vi "RDV-addDataToMap2.vi"(7 "Add mod":string, 8 "error in (no error)":errorcluster, 9 "Data":T1[](array[typedef]), 10 "Names":string[](array[string]), 11 "RDV-Reflection_Data_viewer in":refnum<class "RDV-Reflection_Data_viewer.lvclass">) -> (0 "error out":errorcluster, 1 "Keys":string[](array[string]), 3 "RDV-Reflection_Data_viewer out":refnum<class "RDV-Reflection_Data_viewer.lvclass">)   [LabVIEW 2020, in "RDV-Reflection_Data_viewer.lvclass"]
doc: "Adds data clusters to the viewer's data map, with keys built from the file names and Add mod. Returns the keys."
uses:
  RDV-Reflection_Data_viewer.lvclass
  Reflector/RFH-common_data_format.ctl
  RDV-DATA_MAP_CLUST.ctl
  RDV-Reflection_Data_viewer.lvclass/RDV-Reflection_Data_viewer.ctl
  Reflector/RFH-Reflection_File_Handler.lvlib
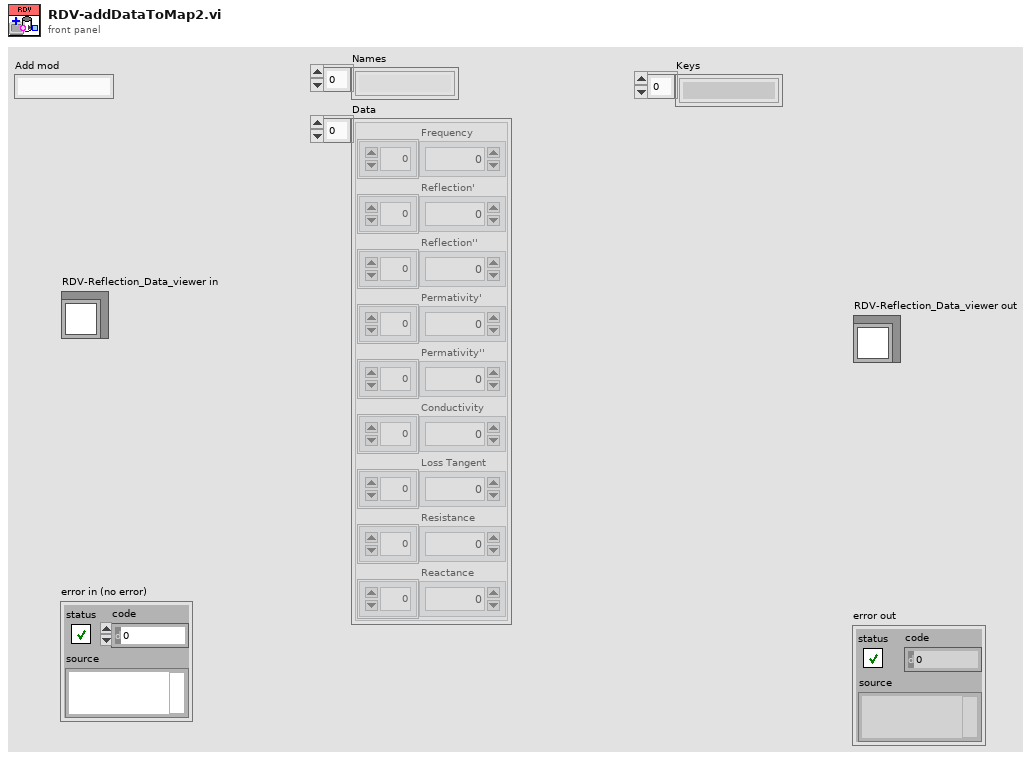
[diagram p1: front panel]
types:
  T1 = typedef "RFH-Reflection_File_Handler.lvlib/RFH-common_data_format.ctl" = cluster{"Frequency":dbl[], "Reflection'":dbl[], "Reflection''":dbl[], "Permativity'":dbl[], "Permativity''":dbl[], "Conductivity":dbl[], "Loss Tangent":dbl[], "Resistance":dbl[], "Reactance":dbl[]}
  T2 = typedef "RDV-Reflection_Data_viewer.lvclass/RDV-DATA_MAP_CLUST.ctl" = cluster{"filename w/ ext":string, "Common Format":T1}
  T3 = typedef "RDV-Reflection_Data_viewer.lvclass/RDV-DATA_MAP.ctl" = map{string, T2}
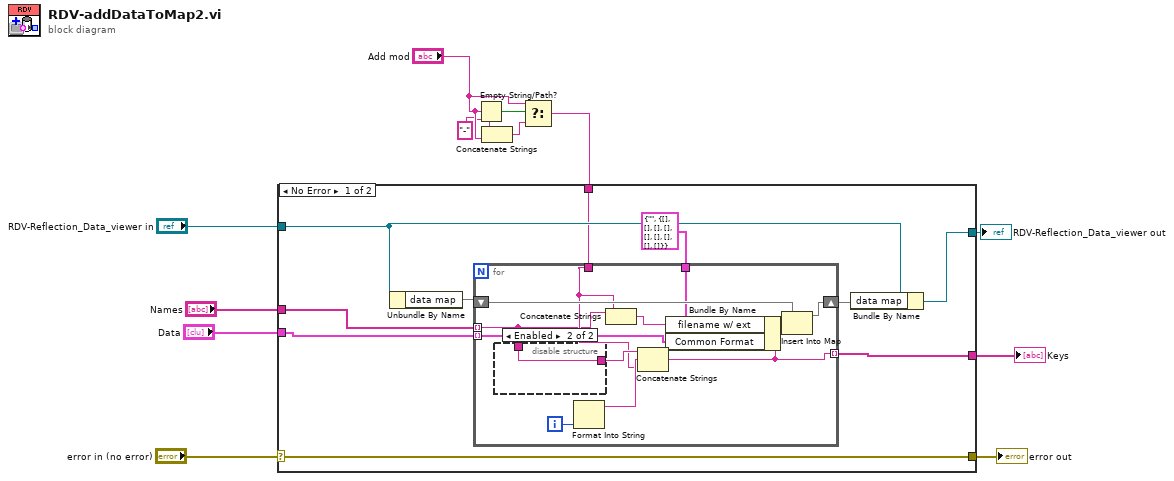
[diagram p0: block diagram]
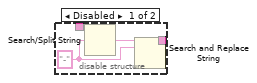
[diagram p2: hidden frame]
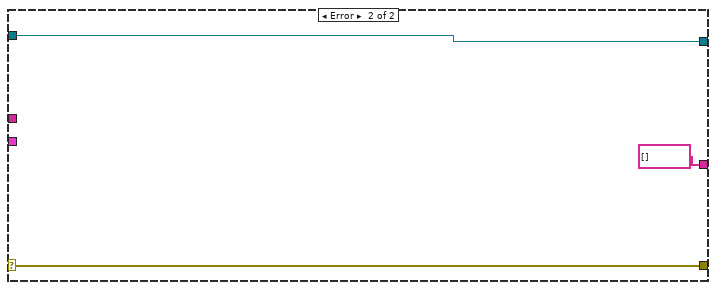
[diagram p3: hidden frame]
diagram:
  n1 = Empty String/Path?(string/path="Add mod") -> (empty?=w6:bool)
  n2 = Concatenate Strings("-" ("string"), "Add mod") -> (w8:string)
  n3 = Select(t="Add mod", s=w6, f=w8) -> (s? t:f=w2:string)
  n4 = case shown="No Error" "error in (no error)" {
    selector: "error in (no error)" -> [w22 w42]
    tunnel: [w22 w42] -> w11
    tunnel: [w16 w41] -> w9
    tunnel: "RDV-Reflection_Data_viewer in" -> [w15 w41]
    tunnel: "Data" -> [w17 _]
    tunnel: "Names" -> [w18 _]
    tunnel: w2 -> [w14 _]
    tunnel: [w13 string[] []] -> w1
    frame No Error {
      n5 = Unbundle By Name(w15) -> ("data map"=w21:T3)
      n6 = for {
        tunnel: w18 -> [w27] mode=indexing
        tunnel: w17 -> [w23] mode=indexing
        shift-right: [w33] -> w20
        shift-left: w21 -> [w34]
        tunnel: [w29] -> w13 mode=indexing
        tunnel: w14 -> [w28]
        tunnel: T2 {"filename w/ ext"="", "Common Format"={"Frequency"=[], "Reflection'"=[], "Reflection''"=[], "Permativity'"=[], "Permativity''"=[], "Conductivity"=[], "Loss Tangent"=[], "Resistance"=[], "Reactance"=[]}} ("map  data") -> [w26]
        i -> [w32]
        n7 = disable-structure shown="Enabled" {
          disable-tunnel: [w36 w39] -> w31
          disable-tunnel: w27 -> [w35 w39]
          frame Disabled {
            w37 = "-" ("search string/char (-)")
            n8 = Search/Split String(string=w35, search string/char (-)=w37) -> (match + rest of string=w38:string)  [unwired: 1 in, 2 out]
            n9 = Search and Replace String(input string=w38, search string=w37) -> (result string=w36:string)  [unwired: 6 in, 3 out]
          }
          frame Enabled {
          }
        }
        n10 = Format Into String(w32) -> (resulting string=w30:string)  [unwired: 3 in, 1 out]
        n11 = Concatenate Strings(w27, w28) -> (w24:string)
        n12 = Concatenate Strings(w31, w30, w28) -> (w29:string)
        n13 = Bundle By Name(cluster=w26, "filename w/ ext"=w24, "Common Format"=w23) -> (w25:T2)
        n14 = Insert Into Map(map in=w34, key=w29, value=w25) -> (map out=w33:T3)  [unwired: 2 out]
      }
      n15 = Bundle By Name(cluster=w15, "data map"=w20) -> (w16:refnum<class "RDV-Reflection_Data_viewer.lvclass">)
    }
    frame Error {
    }
  }
  "error out" <- w11
  "RDV-Reflection_Data_viewer out" <- w9
  "Keys" <- w1
